vi "Post-Install Custom Action.vi"(10 "Variant":variant) -> (0 "error out":errorcluster)   [LabVIEW 2021]
uses:
  <vilib>/Utility/traverseref.llb/TRef TravTarget.ctl
  <vilib>/Utility/traverseref.llb/VI Scripting - Traverse.lvlib
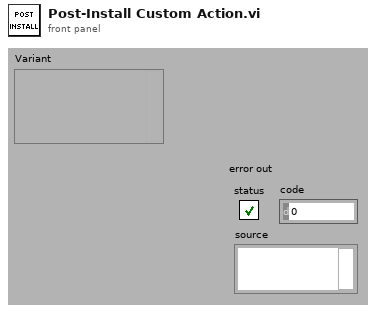
[diagram p1: front panel]
types:
  T1 = typedef "TRef TravTarget.ctl" = enum16{"FP", "BD", "Other"}
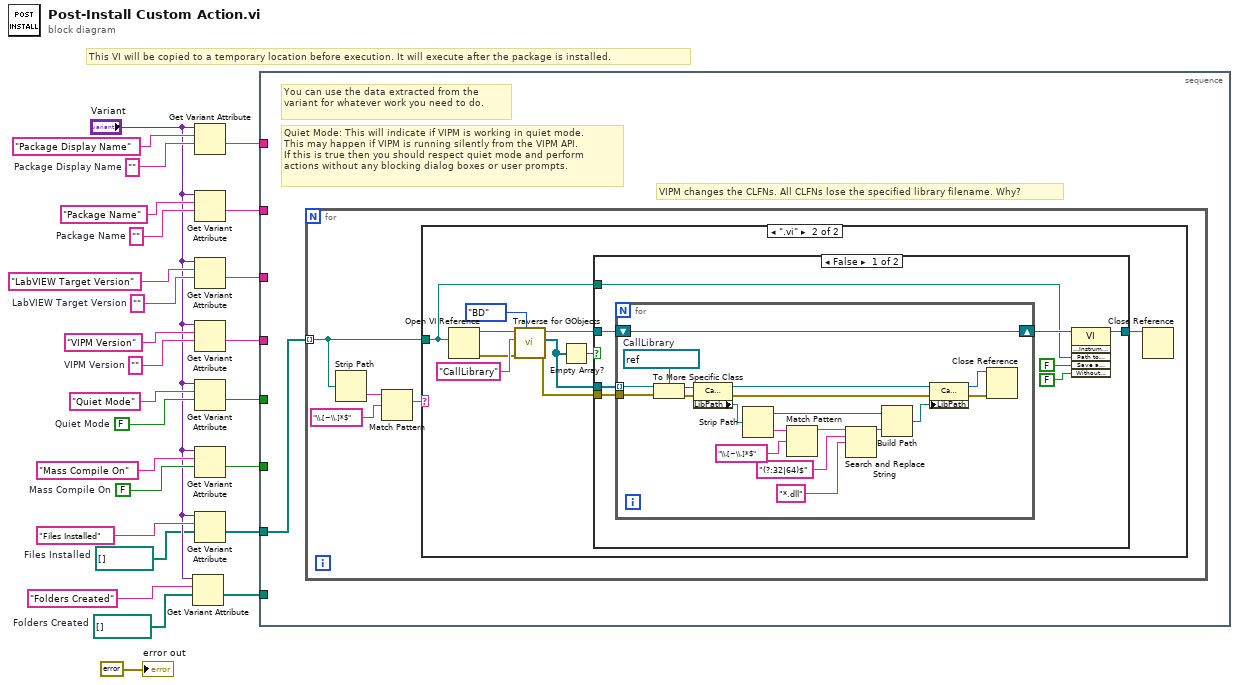
[diagram p0: block diagram]
diagram:
  w2 = path[] []  # Folders Created
  w3 = path[] []  # Files Installed
  w8 = FALSE  # Mass Compile On
  w9 = ""  # Package Display Name
  w16 = FALSE  # Quiet Mode
  w19 = ""  # VIPM Version
  w21 = ""  # LabVIEW Target Version
  w23 = ""  # Package Name
  # "This VI will be copied to a temporary location before execution. It will execute after the package is installed."
  n1 = Get Variant Attribute(Variant="Variant", name="Folders Created", default value (empty Variant)=w2) -> (value=w6:path[])  [unwired: 1 in, 3 out]
  n2 = Get Variant Attribute(Variant="Variant", name="Package Display Name", default value (empty Variant)=w9) -> (value=w15:string)  [unwired: 1 in, 3 out]
  n3 = Get Variant Attribute(Variant="Variant", name="Package Name", default value (empty Variant)=w23) -> (value=w14:string)  [unwired: 1 in, 3 out]
  n4 = Get Variant Attribute(Variant="Variant", name="LabVIEW Target Version", default value (empty Variant)=w21) -> (value=w13:string)  [unwired: 1 in, 3 out]
  n5 = Get Variant Attribute(Variant="Variant", name="VIPM Version", default value (empty Variant)=w19) -> (value=w12:string)  [unwired: 1 in, 3 out]
  n6 = Get Variant Attribute(Variant="Variant", name="Quiet Mode", default value (empty Variant)=w16) -> (value=w11:bool)  [unwired: 1 in, 3 out]
  n7 = Get Variant Attribute(Variant="Variant", name="Mass Compile On", default value (empty Variant)=w8) -> (value=w10:bool)  [unwired: 1 in, 3 out]
  n8 = Get Variant Attribute(Variant="Variant", name="Files Installed", default value (empty Variant)=w3) -> (value=w1:path[])  [unwired: 1 in, 3 out]
  n9 = stacked-sequence {
    tunnel: w15 -> [_]
    tunnel: w14 -> [_]
    tunnel: w13 -> [_]
    tunnel: w12 -> [_]
    tunnel: w11 -> [_]
    tunnel: w10 -> [_]
    tunnel: w1 -> [w27]
    tunnel: w6 -> [_]
    frame #0 {
      # "VIPM changes the CLFNs. All CLFNs lose the specified library filename. Why?"
      # "Quiet Mode: This will indicate if VIPM is working in quiet mode.\nThis may happen if VIPM is running silently from the VIPM API.\nIf this is true then you should respect quiet mode and perform\nactions without any blocking dialog boxes or user prompts."
      # "You can use the data extracted from the variant for whatever work you need to do."
      n10 = for {
        tunnel: w27 -> [w29] mode=indexing
        n11 = Strip Path(path=w29) -> (name=w31:string)  [unwired: 1 out]
        n12 = Match Pattern(string=w31, regular expression="\\.[~\\.]*$") -> (match substring=w28:string)  [unwired: 4 out]
        n13 = case shown="\".vi\"" w28 {
          tunnel: w29 -> [_ w32]
          frame Default {
          }
          frame ".vi" {
            n14 = Open VI Reference(vi path=w32) -> (vi reference=w41:refnum<vi>, error out=w37:errorcluster)  [unwired: 5 in]
            n15 = call <vilib>:"Traverse for GObjects.vi"("Traverse Target"=TRef_TravTarget."BD", "error in (no error)"=w37, "Class Name"="CallLibrary", "VI Refnum"=w41) -> ("error out"=w38:errorcluster, "References"=w34:refnum<vi>[], "dup VI Refnum"=w36:refnum<vi>)  [unwired: 4 in, 1 out]
            n16 = Empty Array?(array=w34) -> (empty?=w33:bool)
            n17 = case shown="False" w33 {
              tunnel: w38 -> [w49 _]
              tunnel: w36 -> [w48 w69]
              tunnel: [w47 w69] -> w35
              tunnel: w34 -> [w46 _]
              tunnel: w32 -> [w43 _]
              frame False {
                n18 = for {
                  tunnel: w46 -> [w51] mode=indexing
                  tunnel: w49 -> [w52]
                  shift-right: [w50] -> w45
                  shift-left: w48 -> [w50]
                  w68 = refnum<vi> refnum  # CallLibrary
                  n19 = To More Specific Class(target class=w68, reference=w51, error in=w52) -> (specific class reference=w67:refnum<vi>, error out=w53:errorcluster)
                  n20 = property class="CallLib"(reference=w67, error in=w53) -> (reference out=w60:refnum<vi>, error out=w54:errorcluster, "LibPath"=w64:path)
                  n21 = Strip Path(path=w64) -> (stripped path=w59:path, name=w66:string)
                  n22 = Match Pattern(string=w66, regular expression="\\.[~\\.]*$") -> (before substring=w63:string)  [unwired: 4 out]
                  n23 = Search and Replace String(input string=w63, search string="(?:32|64)$", replace string="*.dll" ("replace string (\"\")")) -> (result string=w58:string)  [unwired: 5 in, 3 out]
                  n24 = Build Path(base path=w59, name or relative path=w58) -> (appended path=w57:path)
                  n25 = property class="CallLib"(reference=w60, error in=w54, "LibPath"=w57) -> (reference out=w56:refnum<vi>, error out=w55:errorcluster)
                  n26 = Close Reference(reference=w56, error in (no error)=w55) -> ()  [unwired: 1 out]
                }
                n27 = invoke class="VI" method="Save.Instrument"(reference=w45, "Path to saved file"=w43, "Save a Copy"=FALSE, "Without Diagram"=FALSE) -> (reference out=w47:refnum<vi>)  [unwired: 2 in, 5 out]
              }
              frame True {
              }
            }
            n28 = Close Reference(reference=w35) -> ()  [unwired: 1 in, 1 out]
          }
        }
      }
    }
  }
  "error out" <- errorcluster {"status"=FALSE, "code"=0, "source"=""} ("error out")
